vi "Byte_To_SPI_Data.vi"(11 "Byte value":u8) -> (3 "SPI Data":u8[](array[numeric]))   [LabVIEW 2025]
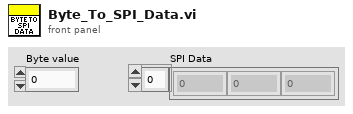
[diagram p1: front panel]
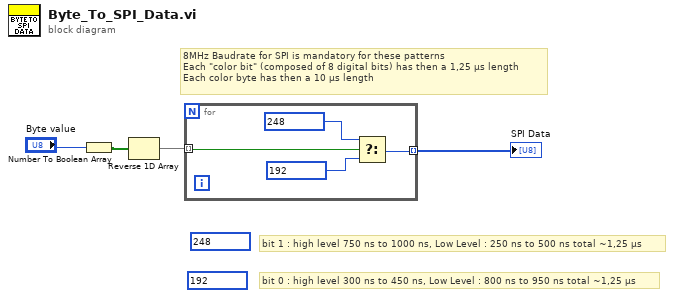
[diagram p0: block diagram]
diagram:
  (unwired) u8 192 ("Numeric")
  (unwired) u8 248 ("Numeric")
  # "bit 1 : high level 750 ns to 1000 ns, Low Level : 250 ns to 500 ns total ~1,25 µs"
  # "bit 0 : high level 300 ns to 450 ns, Low Level : 800 ns to 950 ns total ~1,25 µs"
  # "8MHz Baudrate for SPI is mandatory for these patterns\nEach \"color bit\" (composed of 8 digital bits) has then a 1,25 µs length\nEach color byte has then a 10 µs length"
  n1 = Number To Boolean Array(number="Byte value") -> (Boolean array=w4:bool[])
  n2 = Reverse 1D Array(array=w4) -> (reversed array=w1:bool[])
  n3 = for {
    tunnel: [w5] -> w3 mode=indexing
    tunnel: w1 -> [w7] mode=indexing
    # "GREEN"
    n4 = Select(t=u8 248 ("Numeric"), s=w7, f=u8 192 ("Numeric")) -> (s? t:f=w5:u8)
  }
  "SPI Data" <- w3
